vi "Quick Start - Simple - Create Data Source.vi"   [LabVIEW 2020]
uses:
  Nominal Client/Nominal Client.lvclass/Nominal Client.ctl
  48e63680-6a8c-4ade-94df-21daa40b76be.vi
  Nominal Client/private_data.set.vi
  <vilib>/Utility/file.llb/Application Directory.vi
  <vilib>/Utility/error.llb/Error Cluster From Error Code.vi
  submodules/reqwest-labview/lv-src/reqwest/create.vi
  Nominal Client/Palette Items/who_am_i.vi
  User/User.lvclass
  Nominal Client/Nominal Client.lvclass
  nominal types/workspace/workspace.lvclass
  submodules/reqwest-labview/lv-src/reqwest/reqwest.lvclass
  asset/asset.lvclass
  datasources/dataset/dataset.lvclass
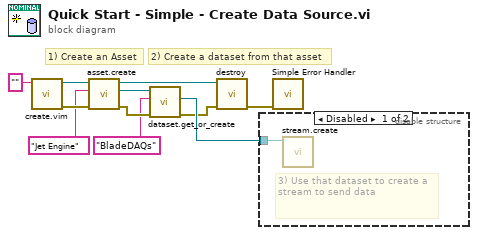
[diagram p0: block diagram]
diagram:
  # "2) Create a dataset from that asset"
  # "1) Create an Asset"
  n1 = call "create.vim"("API Token (string or path)"="") -> ("error out"=w8:errorcluster, "Nominal Client"=w9:refnum<class "Nominal Client.lvclass">)  [unwired: 8 in, 1 out]
  n2 = call "asset.create.vi"("error in"=w8, "Title"="Jet Engine", "Nominal Client in"=w9) -> ("error out"=w6:errorcluster, "asset"=w7:refnum<class "asset.lvclass">, "Nominal Client out"=w1:refnum<class "Nominal Client.lvclass">)  [unwired: 6 in]
  n3 = call "dataset.get_or_create.vi"("error in"=w6, "Datascope Name"="BladeDAQs", "asset in"=w7) -> ("error out"=w2:errorcluster, "dataset"=w3:refnum<class "dataset.lvclass">)  [unwired: 6 in, 1 out]
  n4 = call "destroy.vi"("error in"=w2, "Nominal Client"=w1) -> ("error out"=w10:errorcluster)  [unwired: 9 in]
  n5 = disable-structure shown="Disabled" {
    disable-tunnel: w3 -> [w12 _]
    frame Disabled {
      # "3) Use that dataset to create a stream to send data"
      n6 = call "stream.create.vi"("dataset in"=w12) -> ()  [unwired: 8 in, 3 out]
    }
    frame Enabled {
    }
  }
  n7 = call <vilib>:"Simple Error Handler.vi"("error in (no error)"=w10) -> ()  [unwired: 4 in, 5 out]
